vi "DumpFileCloseFile.vi"(11 "DumpFileState":T1) -> (3 "DumpFileState out":T1)   [LabVIEW 2018]
uses:
  DumpFileState.ctl
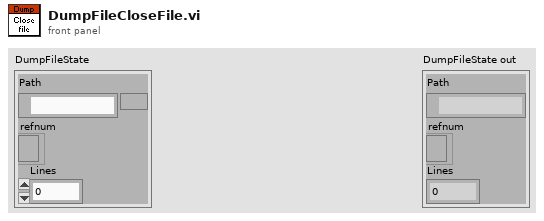
[diagram p1: front panel]
types:
  T1 = typedef "DumpFileState.ctl" = cluster{"Path":path, "refnum":refnum<file>, "Lines":i32}
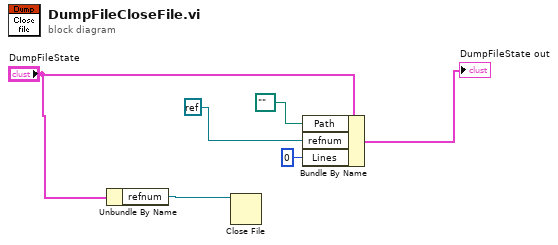
[diagram p0: block diagram]
diagram:
  n1 = Unbundle By Name("DumpFileState") -> ("refnum"=w6:refnum<file>)
  n2 = Close File(refnum=w6) -> ()  [unwired: 1 in, 2 out]
  n3 = Bundle By Name(cluster="DumpFileState", "Path"=path "", "refnum"=refnum<k0> refnum, "Lines"=0) -> (→"DumpFileState out":T1)
